vi "Scaling Params.vi"(8 "error in (no error)":errorcluster, 11 "Scaling in":refnum<class "Scaling Config.lvclass">) -> (0 "error out":errorcluster, 1 "Scale Params":dbl[][](array[numeric]), 2 "Scale Types":T1[](array[typedef]), 3 "Scaling out":refnum<class "Scaling Config.lvclass">)   [LabVIEW 2020, in "VolatusConfig.lvlib" / "Scaling Config.lvclass"]
uses:
  Scaling Config.lvclass
  C:/dev/lv20CE/relink/lv-volatus/VolatusConfig/VolatusConfigElement/VolatusConfigElement.lvclass
  Scale Type.ctl
  Meta Type.ctl
  SensorList/SensorList.lvclass
  Scaling Config.lvclass/Scaling Config.ctl
  VolatusConfigElement/VolatusConfigElement.lvclass/VolatusConfigElement.ctl
  VolatusConfigElement/Element.vi
  lv-cdm/CDM-Config/Config Lookup/Match Meta.vi
  lv-cdm/CDM-Config/Config Element/Owner.vi
  lv-cdm/CDM-Config/Config Manager/Lookup Descendant.vi
  lv-cdm/CDM-Config/Config Filter/Config Lookup.lvclass
  VolatusConfigElement/VolatusConfigElement.lvclass
  VolatusConfig.lvlib
  lv-cdm/CDM-Config/Config Element/Config Element.lvclass
  Scale/Scale Config.lvclass
  VolatusErrorUtilities/MultiErrors/MultiErrors.lvclass
  C:/dev/lv20CE/relink/lv-volatus/VolatusConfig/Scaling/Scaling Config.lvclass
  C:/dev/lv20CE/relink/lv-volatus/VolatusConfig/SensorList/SensorList.lvclass
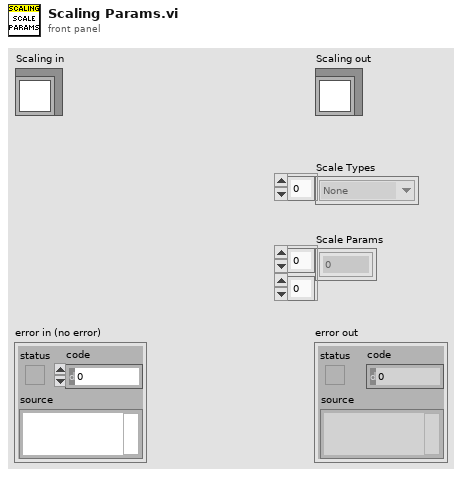
[diagram p1: front panel]
types:
  T1 = typedef "VolatusConfig.lvlib/Scale Type.ctl" = enum16{"None", "Sensor", "Polynomial", "Threshold", "Invert Bool", "Exponential"}
  T2 = typedef "VolatusConfig.lvlib/Meta Type.ctl" = enum16{"UNKNOWN", "VL_System", "VL_Cluster", "VL_Node", "VL_Task", "VL_Group", "VL_Channel", "VL_Task_List", "VL_Scaling", "VL_Sensor", "VL_Sensor_List", "VL_Scale"}
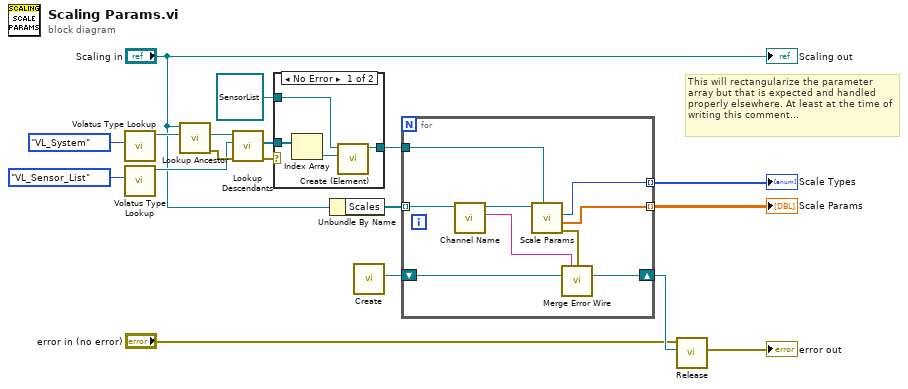
[diagram p0: block diagram]
diagram:
  # "This will rectangularize the parameter array but that is expected and handled properly elsewhere. At least at the time of writing this comment..."
  n1 = call "Volatus Type Lookup.vi"("Meta Type"=Meta_Type."VL_System") -> ("Config Lookup out"=w17:refnum<class "Config Lookup.lvclass">)  [unwired: 9 in, 1 out]
  n2 = call "Volatus Type Lookup.vi"("Meta Type"=Meta_Type."VL_Sensor_List") -> ("Config Lookup out"=w13:refnum<class "Config Lookup.lvclass">)  [unwired: 9 in, 1 out]
  n3 = call "Lookup Ancestor.vi"("Lookup"=w17, "VolatusConfigElement in"="Scaling in") -> ("error out"=w18:errorcluster, "Ancestor"=w14:refnum<class "Config Element.lvclass">)  [unwired: 7 in, 1 out]
  n4 = call "Lookup Descendants.vi"("error in (no error)"=w18, "Lookup"=w13, "Config Element in"=w14) -> ("error out"=w10:errorcluster, "Descendants"=w12:refnum<class "Config Element.lvclass">[])  [unwired: 6 in, 1 out]
  n5 = case shown="No Error" w10 {
    tunnel: w12 -> [w22 _]
    tunnel: refnum<class "SensorList.lvclass"> refnum ("VolatusConfig.lvlib:SensorList.lvclass") -> [w20 w23]
    tunnel: [w19 w23] -> w8
    frame No Error {
      n6 = Index Array(array=w22) -> (element=w21:refnum<class "Config Element.lvclass">)  [unwired: 1 in]
      n7 = call "Create (Element).vi"("Element"=w21, "VolatusConfigElement in"=w20) -> ("VolatusConfigElement out"=w19:refnum<class "SensorList.lvclass">)  [unwired: 8 in, 1 out]
    }
    frame Error {
    }
  }
  n8 = Unbundle By Name("Scaling in") -> ("Scales"=w7:refnum<class "Scale Config.lvclass">[])
  n9 = call "Create.vi"() -> ("MultiErrors out"=w4:refnum<class "MultiErrors.lvclass">)  [unwired: 11 in]
  n10 = for {
    tunnel: w8 -> [w31]
    tunnel: w7 -> [w32] mode=indexing
    tunnel: [w30] -> w5 mode=indexing
    tunnel: [w29] -> w6 mode=indexing
    shift-right: [w26] -> w3
    shift-left: w4 -> [w27]
    n11 = call "Channel Name.vi"("Scale in"=w32) -> ("Channel Name"=w24:string, "Scale out"=w25:refnum<class "Scale Config.lvclass">)  [unwired: 7 in, 2 out]
    n12 = call "Scale Params.vi"("SensorList (Auto)"=w31, "Scale in"=w25) -> ("error out"=w28:errorcluster, "Scale Params"=w29:dbl[], "Scale Type"=w30:T1)  [unwired: 6 in, 1 out]
    n13 = call "Merge Error Wire.vi"("Local Context (None)"=w24, "error in (no error)"=w28, "MultiErrors in"=w27) -> ("MultiErrors out"=w26:refnum<class "MultiErrors.lvclass">)  [unwired: 12 in]
  }
  "Scale Params" <- w6
  "Scale Types" <- w5
  n14 = call "Release.vi"("MultiErrors in"=w3, "Upstream Error (None)"="error in (no error)") -> ("error out"=→"error out":errorcluster)  [unwired: 9 in]
  "Scaling out" <- "Scaling in"
